vi "Decimate DFD (Fs).vi"(6 "Nyquist Filter [F]":bool, 8 "error in (no error)":errorcluster, 9 "output fs (Hz)":dbl=6500.0 format="%#_13g", 10 "Fs":dbl, 11 "Waveforms in":waveform(dbl)[](array[waveform])) -> (0 "error out":errorcluster, 3 "waveforms out":waveform(dbl)[](array[waveform]))   [LabVIEW 2019, in "DSP.lvclass"]
uses:
  DSP.lvclass
  Decimate DFD (Array).vi/949379ad-8373-41eb-be01-93a6c1c1afb3.vi
  Decimate DFD (Array).vi/efb08f77-0c38-4651-8a9c-351b9595fc15.vi
panel:
  out "Decimation Factor":i32
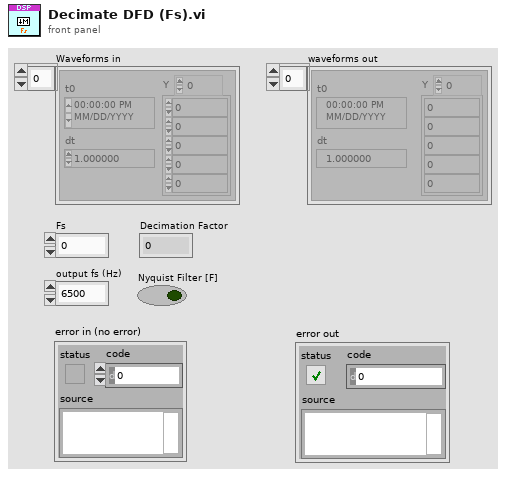
[diagram p1: front panel]
types:
  T1 = cluster{"filter structure":enum32{"IIR 2nd Order", "IIR 4th Order"}, "Reverse Coefficients":dbl[], "Forward Coefficients":dbl[]}[]
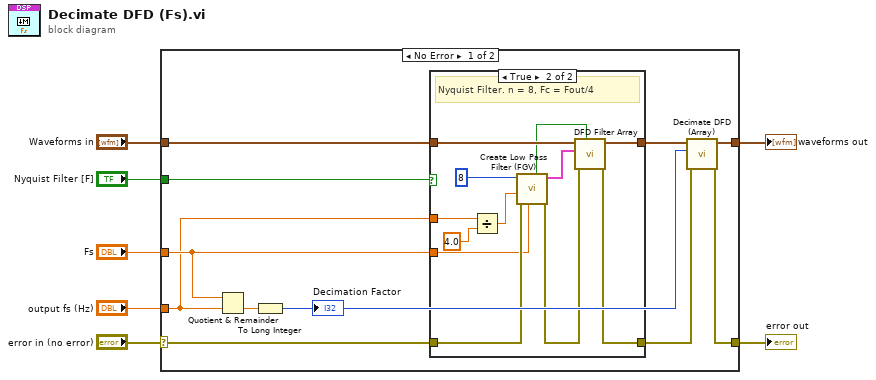
[diagram p0: block diagram]
diagram:
  n1 = case shown="No Error" "error in (no error)" {
    selector: "error in (no error)" -> [w12 w34]
    tunnel: "output fs (Hz)" -> [w9 _]
    tunnel: "Waveforms in" -> [w13 w33]
    tunnel: [w16 w34] -> w4
    tunnel: [w17 w33] -> w3
    tunnel: "Fs" -> [w10 _]
    tunnel: "Nyquist Filter [F]" -> [w8 _]
    frame No Error {
      n2 = Quotient & Remainder(x=w10, y=w9) -> (floor(x/y)=w18:dbl)  [unwired: 1 out]
      n3 = To Long Integer(number=w18) -> (32bit integer=w15:i32)
      "Decimation Factor" <- w15
      n4 = case shown="True" w8 {
        tunnel: [w20 w32] -> w14
        tunnel: w13 -> [w20 w31]
        tunnel: w12 -> [w19 w29]
        tunnel: [w19 w27] -> w11
        tunnel: w10 -> [_ w24]
        tunnel: w9 -> [_ w23]
        frame False {
        }
        frame True {
          # "Nyquist Filter. n = 8, Fc = Fout/4"
          n5 = Divide(x=w23, y=4.0) -> (x/y=w21:dbl)
          n6 = call "Create Low Pass Filter (FGV).vi"("fs (Hz)"=w24, "error in (no error)"=w29, "Low Pass Cutoff (Hz)"=w21, "order"=8) -> ("error out"=w28:errorcluster, "IIR Filters"=w25:T1, "init out"=w30:bool)  [unwired: 5 in]
          n7 = call "DFD Filter Array.vi"("init (F)"=w30, "error in (no error)"=w28, "IIR Filters"=w25, "signal in"=w31) -> ("error out"=w27:errorcluster, "signal out"=w32:waveform(dbl)[])  [unwired: 6 in]
        }
      }
      n8 = call "Decimate DFD (Array).vi"("error in (no error)"=w11, "Decimation Factor"=w15, "Waveforms in"=w14) -> ("error out"=w16:errorcluster, "waveforms out"=w17:waveform(dbl)[])  [unwired: 7 in]
    }
    frame Error {
    }
  }
  "waveforms out" <- w3
  "error out" <- w4
